vi "Calculate Common Root.vi"(8 "error in (no error)":errorcluster, 10 "Generated Files":path[](array[path])) -> (0 "error out":errorcluster, 2 "Root Path":path)   [LabVIEW 2014, in "G CLI LvBuild.lvlib"]
uses:
  G CLI LvBuild.lvlib
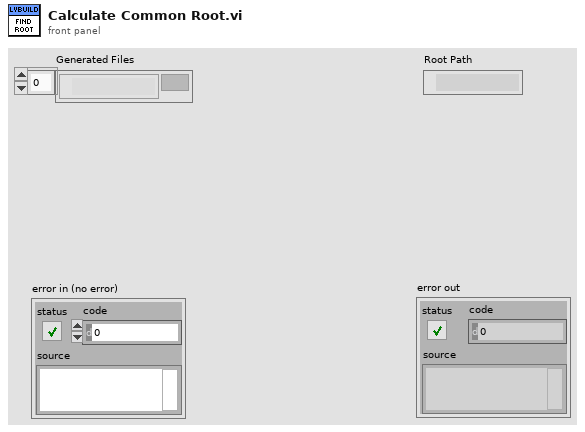
[diagram p1: front panel]
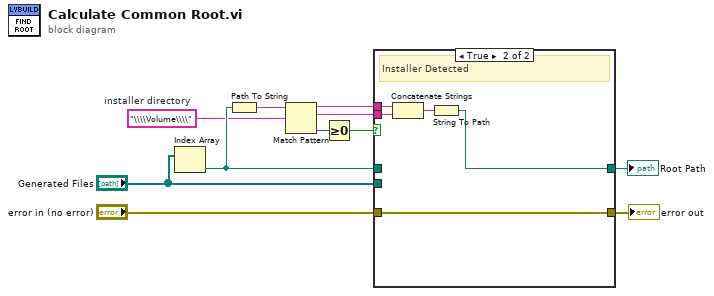
[diagram p0: block diagram]
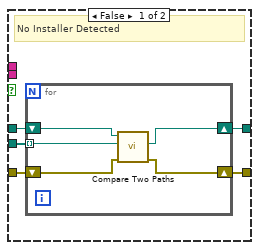
[diagram p2: hidden frame]
diagram:
  w5 = "\\\\Volume\\\\"  # installer directory
  n1 = Index Array(array="Generated Files") -> (element=w7:path)  [unwired: 1 in]
  n2 = Path To String(path=w7) -> (string=w6:string)
  n3 = Match Pattern(string=w6, regular expression=w5) -> (before substring=w2:string, match substring=w1:string, offset past match=w4:i32)  [unwired: 1 in, 1 out]
  n4 = Greater Or Equal To 0?(x=w4) -> (x >= 0?=w3:bool)
  n5 = case shown="True" w3 {
    tunnel: "Generated Files" -> [w16 _]
    tunnel: [w15 w23] -> w10
    tunnel: "error in (no error)" -> [w14 w22]
    tunnel: [w13 w22] -> w8
    tunnel: w7 -> [w12 _]
    tunnel: w2 -> [_ w26]
    tunnel: w1 -> [_ w25]
    frame False {
      # "No Installer Detected"
      n6 = for {
        tunnel: w16 -> [w21] mode=indexing
        shift-right: [w19] -> w15
        shift-left: w12 -> [w20]
        shift-right: [w17] -> w13
        shift-left: w14 -> [w18]
        n7 = call <vilib>:"Compare Two Paths.vi"("error in (no error)"=w18, "Path 2"=w21, "Path 1"=w20) -> ("error out"=w17:errorcluster, "Common Path"=w19:path)  [unwired: 5 in, 2 out]
      }
    }
    frame True {
      # "Installer Detected"
      n8 = Concatenate Strings(w26, w25) -> (w24:string)
      n9 = String To Path(string=w24) -> (path=w23:path)
    }
  }
  "Root Path" <- w10
  "error out" <- w8
